vi "UDPEngine.Main.vi"(7 "WaveformChart Ref":refnum<vi>, 8 "error in (no error)":errorcluster, 9 "ClientPort":u16, 10 "UDP Engine Queue":refnum<queue>, 11 "WorkspaceManager":T1) -> (0 "error out":errorcluster, 1 "Exit":bool, 2 "Update?":bool, 3 "Waveform":waveform(dbl)[](array[waveform]))   [LabVIEW 2015, in "Single Station Execution.lvlib"]
uses:
  Single Station Execution.lvlib
  Types/UDPEngine.QueueCluster.ctl
  Types/UDPEngine.State.ctl
  <vilib>/NI Veristand/Execution/Workspace/WorkspaceAPI.ctl
  NationalInstruments.VeriStand.ClientAPI
  <vilib>/NI Veristand/Execution/Workspace/UDPChannelStreamSession.ctl
  NationalInstruments.VeriStand
  <vilib>/NI Veristand/Execution/Workspace/UDP Stream Packet.ctl
  <vilib>/Utility/tcp.llb/UDP Multicast Read-Only Open.vi
  <vilib>/NI Veristand/Execution/Workspace/NI_VS Workspace ExecutionAPI.lvlib
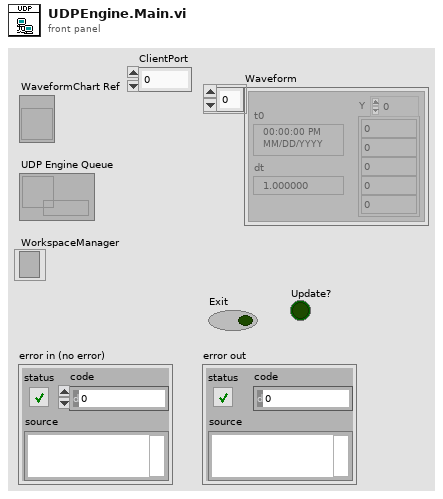
[diagram p1: front panel]
types:
  T1 = typedef "NI_VS Workspace ExecutionAPI.lvlib/WorkspaceAPI.ctl" = refnum<k24>
  T2 = typedef "Single Station Execution.lvlib/UDPEngine.State.ctl" = enum8{"Idle", "Start Acq", "Run", "Stop Acq", "Exit"}
  T3 = typedef "NI_VS Workspace ExecutionAPI.lvlib/UDPChannelStreamSession.ctl" = refnum<k24>
  T4 = cluster{"Initialized Waveform":waveform(dbl)[], "VS UDP Session":T3, "Channel IDs":i32[], "Packet IDs":i32[], "Max Packet Size":i32, "UDP Ref":refnum<k16>}
  T5 = typedef "Single Station Execution.lvlib/UDPEngine.QueueCluster.ctl" = cluster{"Action":T2, "Channels":string[]}
  T6 = typedef "NI_VS Workspace ExecutionAPI.lvlib/UDP Stream Packet.ctl" = cluster{"ID":i32, "t0":dbl, "dt":dbl, "Channel IDs":i32[], "Channel Data":dbl[][], "Sample Offset":u64}
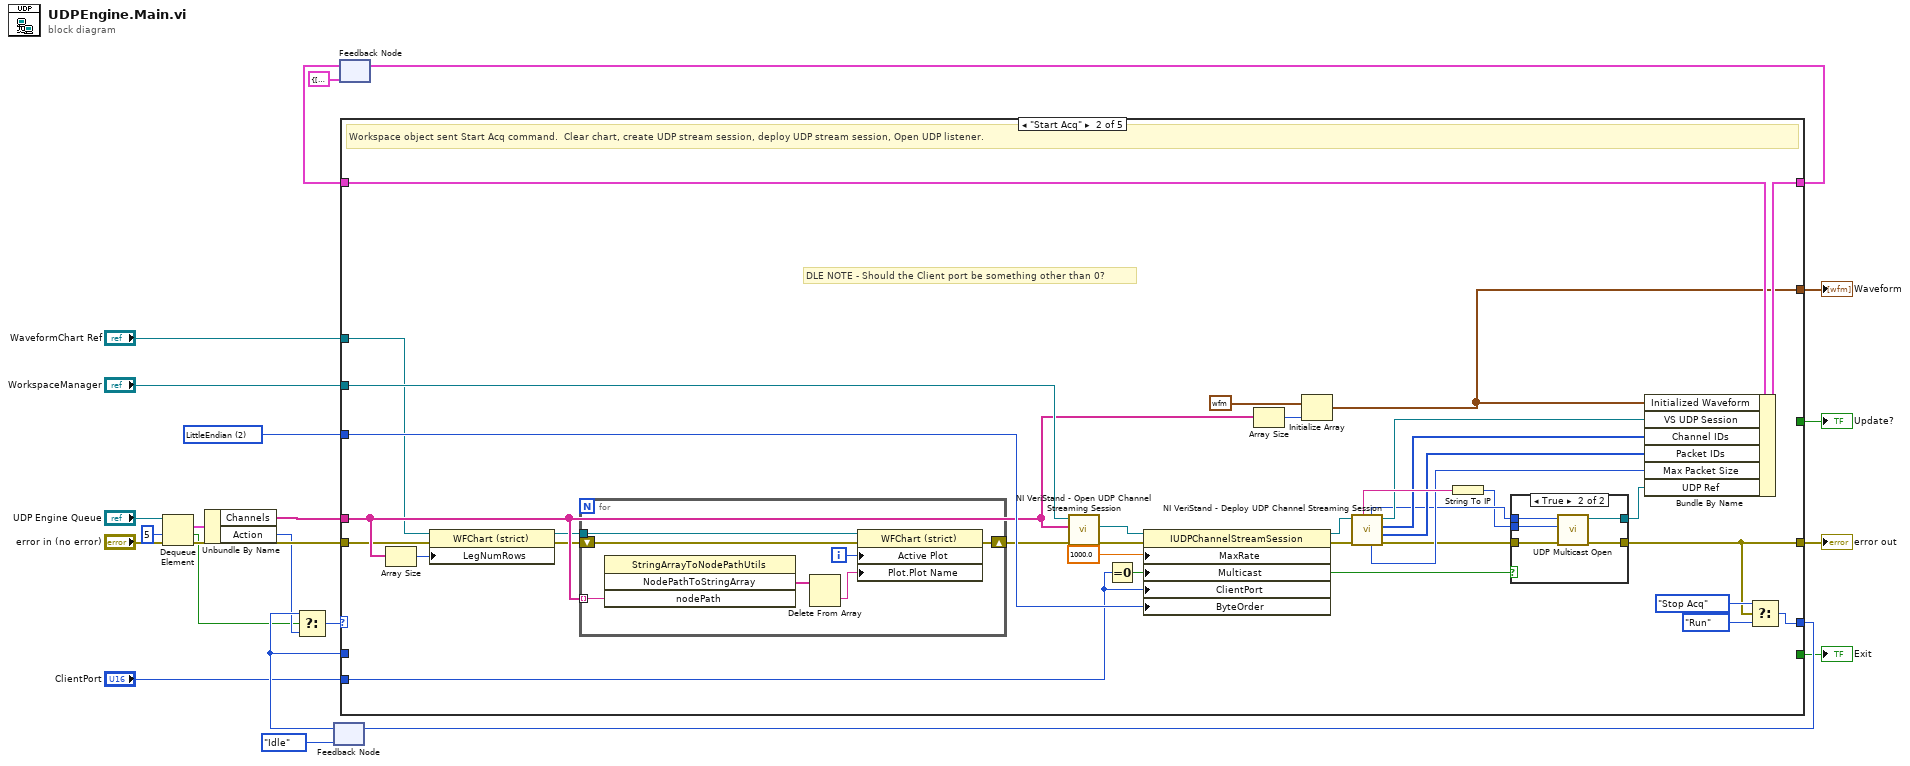
[diagram p0: block diagram]
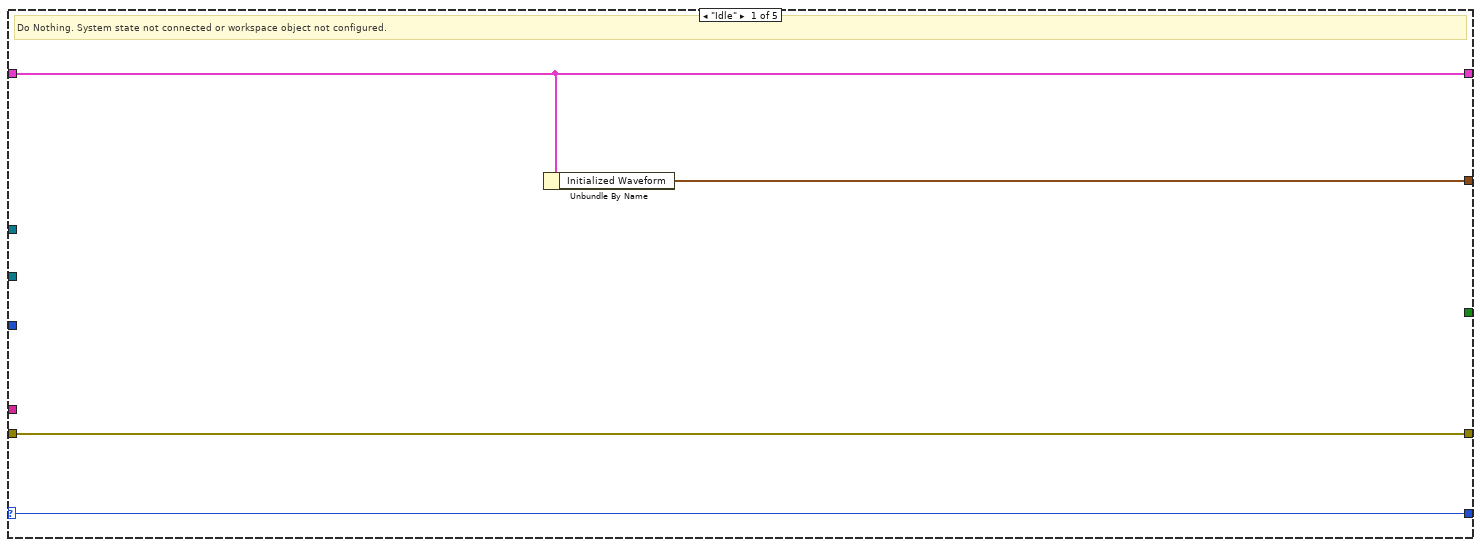
[diagram p2: hidden frame]
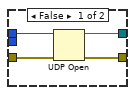
[diagram p3: hidden frame]
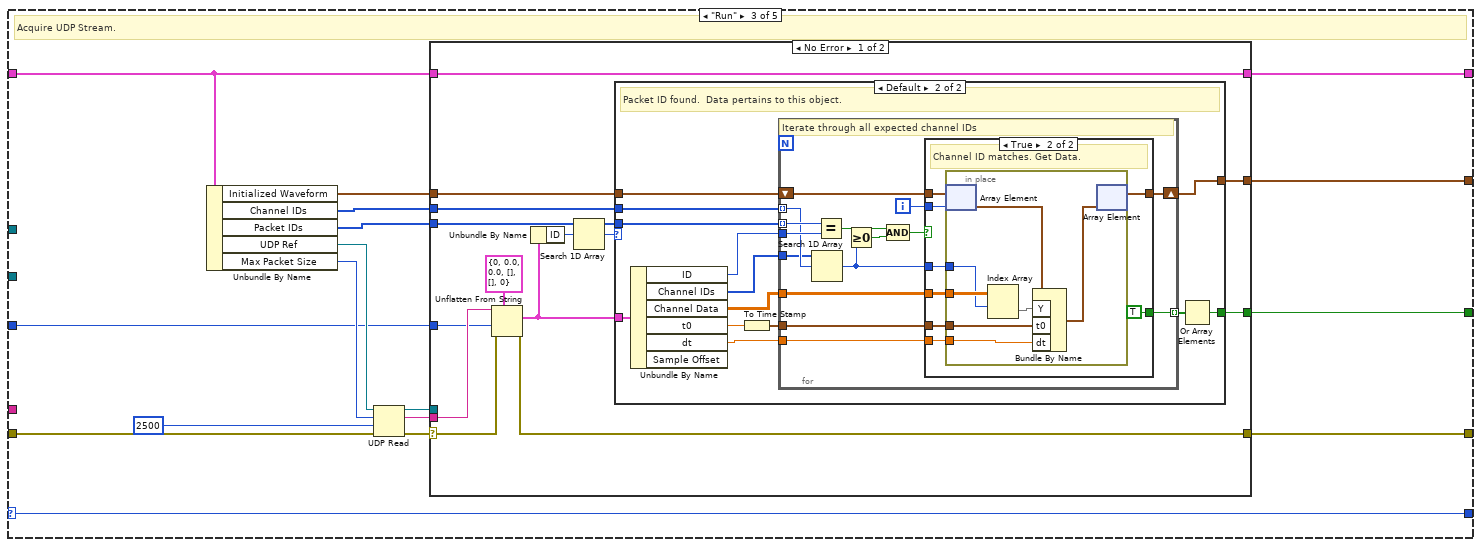
[diagram p4: hidden frame]
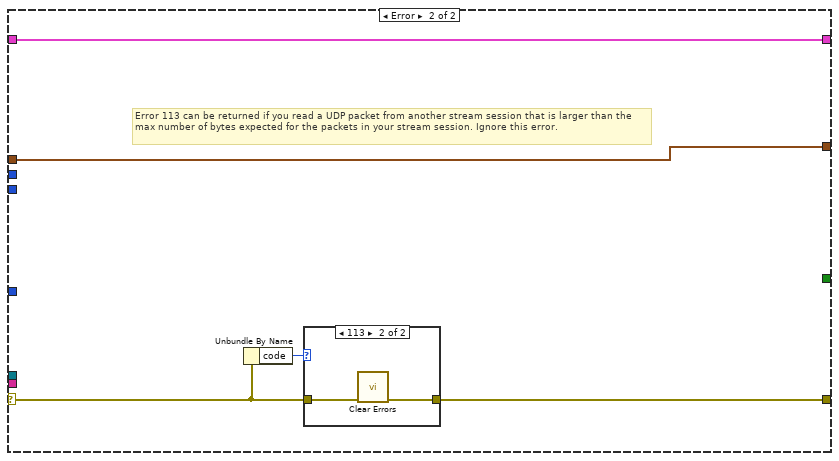
[diagram p7: hidden frame]
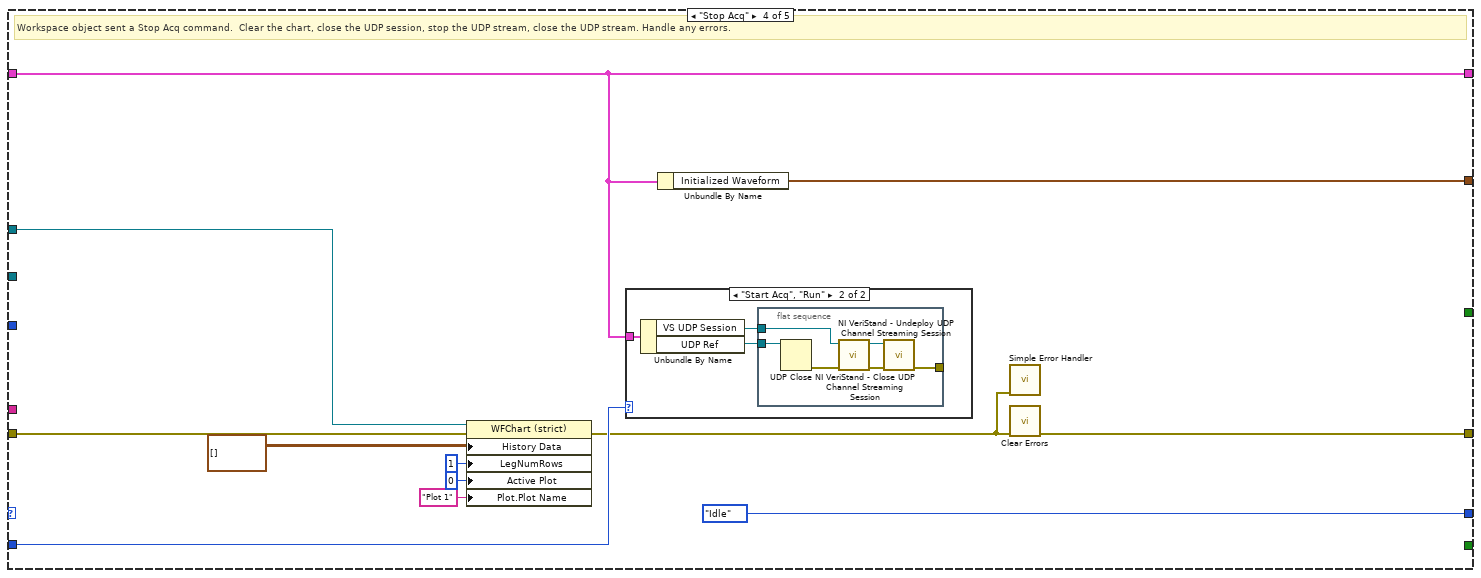
[diagram p9: hidden frame]
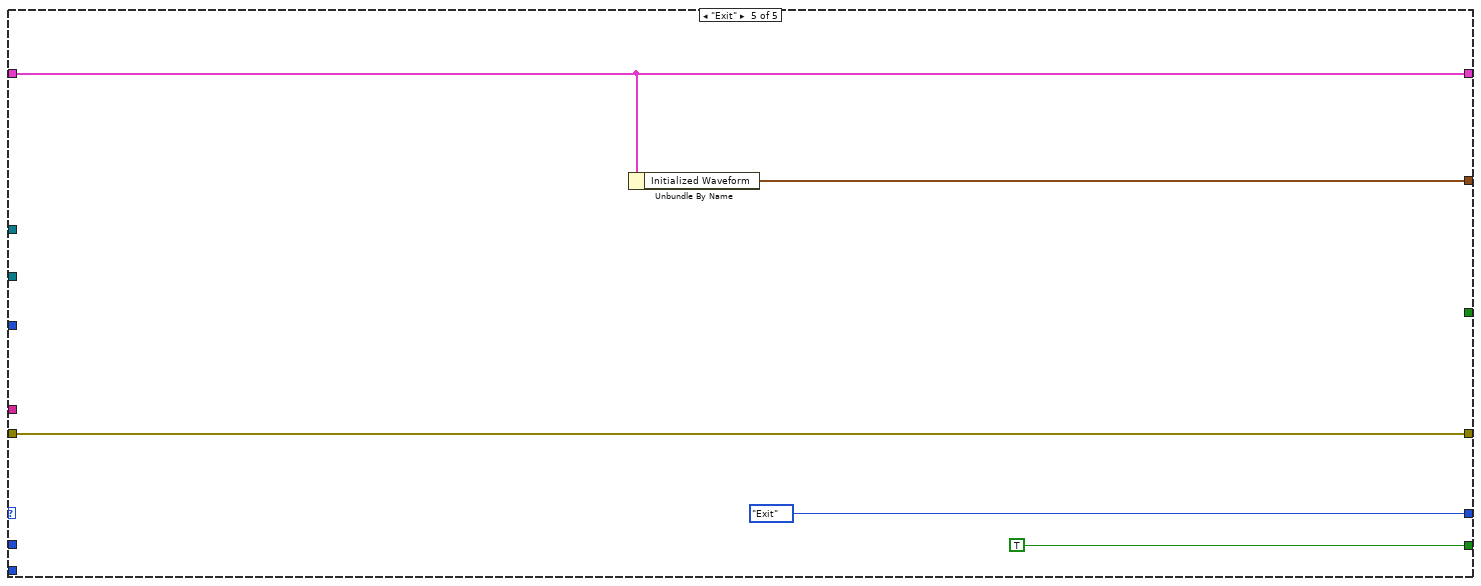
[diagram p11: hidden frame]
diagram:
  w17 = 2 items=["BigEndian", "NativeHostOrder", "LittleEndian"] ("Byte Order")
  n1 = Dequeue Element(queue="UDP Engine Queue", timeout in ms (-1)=5, error in (no error)="error in (no error)") -> (element=w7:T5, timed out?=w9:bool, error out=w13:errorcluster)  [unwired: 1 out]
  n2 = Unbundle By Name(w7) -> ("Channels"=w16:string[], "Action"=w10:T2)
  n3 = feedback #1(UDPEngine.State."Idle" ("Action")) -> (w22:T2)
  n4 = Select(t=w22, s=w9, f=w10) -> (s? t:f=w11:T2)
  n5 = feedback #2(T4 {"Initialized Waveform"=[], "VS UDP Session"=refnum, "Channel IDs"=[], "Packet IDs"=[], "Max Packet Size"=0, "UDP Ref"=refnum}) -> (w19:T4)
  n6 = case shown="\"Start Acq\"" w11 {
    selector: w11 -> [w26 _ w83 _ _]
    tunnel: "WorkspaceManager" -> [_ w53 _ _ _]
    tunnel: w19 -> [w25 w52 w84 w167 w185]
    tunnel: w17 -> [_ w48 w80 _ _]
    tunnel: [w25 w47 w85 w167 w185] -> w18
    tunnel: [w26 w46 w83 UDPEngine.State."Idle" ("Action") UDPEngine.State."Exit" ("Action")] -> w21
    tunnel: [_ _ _ _ TRUE] -> w12
    tunnel: w13 -> [w27 w39 w82 w169 w186]
    tunnel: [w27 w30 w81 w173 w186] -> w14
    tunnel: w16 -> [_ w41 _ _ _]
    tunnel: w22 -> [_ _ _ w172 _]
    tunnel: [w24 w45 w79 w166 w184] -> w23
    tunnel: "WaveformChart Ref" -> [_ w40 _ w171 _]
    tunnel: [_ _ w78 _ _] -> w4
    tunnel: "ClientPort" -> [_ w34 _ _ _]
    frame "Idle" {
      # "Do Nothing. System state not connected or workspace object not configured."
      n7 = Unbundle By Name(w25) -> ("Initialized Waveform"=w24:waveform(dbl)[])
    }
    frame "Start Acq" {
      # "DLE NOTE - Should the Client port be something other than 0?"
      # "Workspace object sent Start Acq command.  Clear chart, create UDP stream session, deploy UDP stream session, Open UDP listener."
      n8 = Array Size(array=w41) -> (size(s)=w36:i32)
      n9 = property on="Property Node" class="WFChart (strict)"(reference=w40, error in=w39, "LegNumRows"=w36) -> (reference out=w37:refnum<vi>, error out=w38:errorcluster)
      n10 = for {
        tunnel: w37 -> [w77]
        shift-right: [w75] -> w42
        shift-left: w38 -> [w76]
        tunnel: w41 -> [w73] mode=indexing
        i -> [w74]
        n11 = invoke class="StringArrayToNodePathUtils" method="NodePathToStringArray"("nodePath"=w73) -> ("NodePathToStringArray"=w72:string[])  [unwired: 3 in, 3 out]
        n12 = Delete From Array(array=w72) -> (deleted portion=w71:string)  [unwired: 2 in, 1 out]
        n13 = property on="Property Node" class="WFChart (strict)"(reference=w77, error in=w76, "Active Plot"=w74, "Plot.Plot Name"=w71) -> (error out=w75:errorcluster)  [unwired: 1 out]
      }
      n14 = call <vilib>:"NI VeriStand - Open UDP Channel Streaming Session.vi"("error in (no error)"=w42, "Channels"=w41, "WorkspaceManager in"=w53) -> ("error out"=w60:errorcluster, "UDPChannelStreamSession out"=w57:T3)  [unwired: 6 in, 1 out]
      n15 = Equal To 0?(x=w34) -> (x = 0?=w29:bool)
      n16 = property class="IUDPChannelStreamSession"(reference=w57, error in=w60, "MaxRate"=1000.0, "Multicast"=w29, "ClientPort"=w34, "ByteOrder"=w48) -> (reference out=w59:T3, error out=w58:errorcluster)
      n17 = Array Size(array=w41) -> (size(s)=w55:i32)
      n18 = Initialize Array(waveform(dbl) {"t0"=timestamp(0 s since 1904-01-01), "dt"=1.0, "Y"=[]}, w55) -> (w45:waveform(dbl)[])
      n19 = call <vilib>:"NI VeriStand - Deploy UDP Channel Streaming Session.vi"("error in (no error)"=w58, "UDPChannelStreamSession in"=w59) -> ("error out"=w31:errorcluster, "Packet IDs"=w49:i32[], "Channel IDs"=w50:i32[], "UDPChannelStreamSession out"=w51:T3, "Max Packet Size"=w35:i32, "Port"=w33:u16, "UDP Multicast Address"=w54:string)  [unwired: 3 in]
      n20 = String To IP(1:w54) -> (0:w32:u32)
      n21 = case shown="True" w29 {
        tunnel: w31 -> [w64 w70]
        tunnel: w33 -> [w65 w69]
        tunnel: w32 -> [_ w68]
        tunnel: [w63 w66] -> w28
        tunnel: [w62 w67] -> w30
        frame False {
          n22 = UDP Open(8:w64, 11:w65) -> (port=w63:refnum<k16>, 0:w62:errorcluster)  [unwired: 3 in, 1 out]
        }
        frame True {
          n23 = call-poly <vilib>:"UDP Multicast Open.vi"("error in (no error)"=w70, "multicast addr"=w68, "port"=w69) -> ("error out"=w67:errorcluster, "connection ID"=w66:refnum<k16>)  [unwired: 6 in, 1 out]
        }
      }
      n24 = Bundle By Name(cluster=w52, "Initialized Waveform"=w45, "VS UDP Session"=w51, "Channel IDs"=w50, "Packet IDs"=w49, "Max Packet Size"=w35, "UDP Ref"=w28) -> (w47:T4)
      n25 = Select(t=UDPEngine.State."Stop Acq" ("Action"), s=w30, f=UDPEngine.State."Run" ("Action")) -> (s? t:f=w46:T2)
    }
    frame "Run" {
      # "Acquire UDP Stream."
      n26 = Unbundle By Name(w84) -> ("Initialized Waveform"=w90:waveform(dbl)[], "Channel IDs"=w89:i32[], "Packet IDs"=w88:i32[], "UDP Ref"=w87:refnum<k16>, "Max Packet Size"=w86:i32)
      n27 = UDP Read(connection ID=w87, max size (548)=w86, timeout ms (25000)=2500, 8:w82) -> (data out=w92:string, error out=w93:errorcluster, 3:w94:refnum<k16>)  [unwired: 2 out]
      n28 = case shown="No Error" w93 {
        selector: w93 -> [w107 w155]
        tunnel: w88 -> [w102 _]
        tunnel: w92 -> [w105 _]
        tunnel: w89 -> [w104 _]
        tunnel: w90 -> [w103 w156]
        tunnel: [w108 w157] -> w81
        tunnel: w94 -> [_ _]
        tunnel: w80 -> [w98 _]
        tunnel: [w97 w158] -> w85
        tunnel: w84 -> [w97 w158]
        tunnel: [w96 w156] -> w79
        tunnel: [w95 _] -> w78
        frame No Error {
          n29 = Unflatten From String(type=T6 {"ID"=0, "t0"=0.0, "dt"=0.0, "Channel IDs"=[], "Channel Data"=[], "Sample Offset"=0} ("UDP Data Packet"), binary string=w105, byte order (0:big-endian, network order)=w98, error in (no error)=w107) -> (value=w99:T6, error out=w108:errorcluster)  [unwired: 1 in, 1 out]
          n30 = Unbundle By Name(w99) -> ("ID"=w100:i32)
          n31 = Search 1D Array(1D array=w102, element=w100) -> (index of element=w101:i32)  [unwired: 1 in]
          n32 = case shown="Default" w101 {
            tunnel: w104 -> [_ w122]
            tunnel: w103 -> [w109 w121]
            tunnel: w102 -> [_ w119]
            tunnel: w99 -> [_ w118]
            tunnel: [w109 w112] -> w96
            tunnel: [_ w110] -> w95
            frame -1 {
              # "This is a packet from a different UDP session. Ignore it."
            }
            frame Default {
              # "Packet ID found.  Data pertains to this object."
              n33 = Unbundle By Name(w118) -> ("ID"=w117:i32, "Channel IDs"=w116:i32[], "Channel Data"=w115:dbl[][], "t0"=w114:dbl, "dt"=w113:dbl)  [unwired: 1 out]
              n34 = To Time Stamp(1:w114) -> (0:w120:timestamp)
              n35 = for {
                tunnel: w122 -> [w135] mode=indexing
                tunnel: w119 -> [w137] mode=indexing
                tunnel: w117 -> [w136]
                tunnel: w115 -> [w129]
                tunnel: w116 -> [w128]
                shift-right: [w124] -> w112
                shift-left: w121 -> [w127]
                tunnel: w120 -> [w126]
                tunnel: w113 -> [w125]
                tunnel: [w123] -> w111 mode=indexing
                i -> [w130]
                # "Iterate through all expected channel IDs"
                n36 = Search 1D Array(1D array=w128, element=w135) -> (index of element=w131:i32)  [unwired: 1 in]
                n37 = Equal?(x=w137, y=w136) -> (x = y?=w134:bool)
                n38 = Greater Or Equal To 0?(x=w131) -> (x >= 0?=w133:bool)
                n39 = Compound Arithmetic op=AND(w134, w133) -> (w132:bool)
                n40 = case shown="True" w132 {
                  tunnel: w131 -> [_ w144]
                  tunnel: w130 -> [_ w140]
                  tunnel: w129 -> [_ w145]
                  tunnel: w127 -> [w138 w146]
                  tunnel: w126 -> [_ w143]
                  tunnel: w125 -> [_ w142]
                  tunnel: [w138 w141] -> w124
                  tunnel: [_ TRUE] -> w123
                  frame False {
                    # "This channel is not in this UDP Data Packet."
                  }
                  frame True {
                    # "Channel ID matches. Get Data."
                    n41 = in-place {
                      in-place-border: w145 -> [w152]
                      in-place-border: w144 -> [w151]
                      in-place-border: w143 -> [w149]
                      in-place-border: w142 -> [w148]
                      n42 = in-place-array #3(w146, w140) -> (w153:waveform(dbl))
                      n43 = Index Array(array=w152, index (row)=w151) -> (element=w150:dbl[])  [unwired: 1 in]
                      n44 = Bundle By Name(cluster=w153, "Y"=w150, "t0"=w149, "dt"=w148) -> (w147:waveform(dbl))
                      n45 = in-place-array #3(w147) -> (w141:waveform(dbl)[])  [unwired: 1 out]
                    }
                  }
                }
              }
              n46 = Or Array Elements(Boolean array=w111) -> (logical OR=w110:bool)
            }
          }
        }
        frame Error {
          # "Error 113 can be returned if you read a UDP packet from another stream session that is larger than the max number of bytes expected for the packets in your stream session. Ignore this error."
          n47 = Unbundle By Name(w155) -> ("code"=w154:i32)
          n48 = case shown="113" w154 {
            tunnel: [w159 w161] -> w157
            tunnel: w155 -> [w159 w160]
            frame Default {
            }
            frame 113 {
              n49 = call <vilib>:"Clear Errors.vi"("error in (no error)"=w160) -> ("error out"=w161:errorcluster)  [unwired: 5 in, 1 out]
            }
          }
        }
      }
    }
    frame "Stop Acq" {
      # "Workspace object sent a Stop Acq command.  Clear the chart, close the UDP session, stop the UDP stream, close the UDP stream. Handle any errors."
      n50 = property on="Property Node" class="WFChart (strict)"(reference=w171, error in=w169, "History Data"=waveform(dbl)[][] [], "LegNumRows"=u32 1 ("Legend:Number of Rows"), "Active Plot"=u32 0, "Plot.Plot Name"="Plot 1") -> (error out=w168:errorcluster)  [unwired: 1 out]
      n51 = case shown="\"Start Acq\", \"Run\"" w172 {
        tunnel: w167 -> [_ w174]
        frame Default {
        }
        frame "Start Acq", "Run" {
          n52 = Unbundle By Name(w174) -> ("VS UDP Session"=w175:T3, "UDP Ref"=w176:refnum<k16>)
          n53 = flat-sequence {
            tunnel: w176 -> [w179]
            tunnel: w175 -> [w178]
            tunnel: [w177] -> _
            frame #0 {
              n54 = UDP Close(connection ID=w179) -> (error out=w182:errorcluster)  [unwired: 1 in, 1 out]
              n55 = call <vilib>:"NI VeriStand - Undeploy UDP Channel Streaming Session.vi"("error in (no error)"=w182, "UDPChannelStreamSession in"=w178) -> ("error out"=w180:errorcluster, "UDPChannelStreamSession out"=w181:T3)  [unwired: 8 in]
              n56 = call <vilib>:"NI VeriStand - Close UDP Channel Streaming Session.vi"("error in (no error)"=w180, "UDPChannelStreamSession in"=w181) -> ("error out"=w177:errorcluster)  [unwired: 9 in]
            }
          }
        }
      }
      n57 = Unbundle By Name(w167) -> ("Initialized Waveform"=w166:waveform(dbl)[])
      n58 = call <vilib>:"Simple Error Handler.vi"("error in (no error)"=w168) -> ()  [unwired: 4 in, 5 out]
      n59 = call <vilib>:"Clear Errors.vi"("error in (no error)"=w168) -> ("error out"=w173:errorcluster)  [unwired: 5 in, 1 out]
    }
    frame "Exit" {
      n60 = Unbundle By Name(w185) -> ("Initialized Waveform"=w184:waveform(dbl)[])
    }
  }
  "Waveform" <- w23
  "error out" <- w14
  "Exit" <- w12
  "Update?" <- w4
  n61 = feedback-in #1(w21) -> ()
  n62 = feedback-in #2(w18) -> ()
